vi "DSS-Tests-golden_write.vi"(8 "error in":errorcluster, 10 "values":dbl[](array[numeric]), 11 "file path":path) -> (0 "error out":errorcluster)   [LabVIEW 2020, in "DSS-Tests.lvlib"]
doc: "Writes a 1D DBL array to a golden text file, one value per line with %.16e and a period as decimal point so the text reads back exactly, creating the folder if needed."
uses:
  DSS-Tests.lvlib
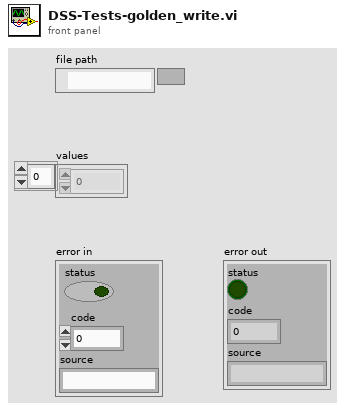
[diagram p1: front panel]
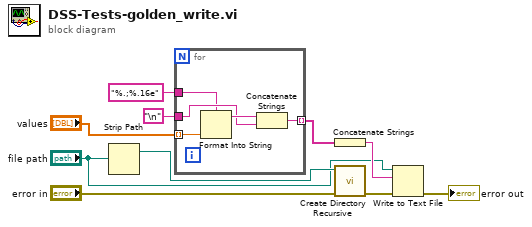
[diagram p0: block diagram]
diagram:
  n1 = Strip Path(path="file path") -> (stripped path=w4:path)  [unwired: 1 out]
  n2 = for {
    tunnel: "values" -> [w11] mode=indexing
    tunnel: "%.;%.16e" ("format string") -> [w12]
    tunnel: "\n" ("Line Feed Constant") -> [w13]
    tunnel: [w15] -> w8 mode=indexing
    n3 = Format Into String(format string=w12, w11) -> (resulting string=w14:string)  [unwired: 2 in, 1 out]
    n4 = Concatenate Strings(w14, w13) -> (w15:string)
  }
  n5 = Concatenate Strings(w8) -> (w9:string)
  n6 = call <vilib>:"Create Directory Recursive.vi"("error in (no error)"="error in", "directory"=w4) -> ("error out"=w5:errorcluster)  [unwired: 3 in, 2 out]
  n7 = Write to Text File(file (use dialog)="file path", text=w9, error in=w5) -> (error out=→"error out":errorcluster)  [unwired: 1 in, 2 out]
